vi "mupSetLocale.vi"(8 "error in (no error)":errorcluster, 10 "Use system decimal point (T)":bool=TRUE, 11 "hParser in":u64) -> (0 "error out":errorcluster, 3 "hParser out":u64)   [LabVIEW 2018, in "mupLib.lvlib"]
doc: "Set to true to use system's decimal point.\n\nIf the system's decimal point is a comma, the argument separator will be changed to a semi-colon.\n\nThe default decimal point is a period. The default argument separator is a comma."
uses:
  mupLib.lvlib
  libmuparser-lv.dll
panel:
  # "Set to true to use system's decimal point.\n\nIf the system's decimal point is a comma, the argument separator will be changed to a semi-colon.\n\nThe default decimal point is a period. The default argument separator is a comma."
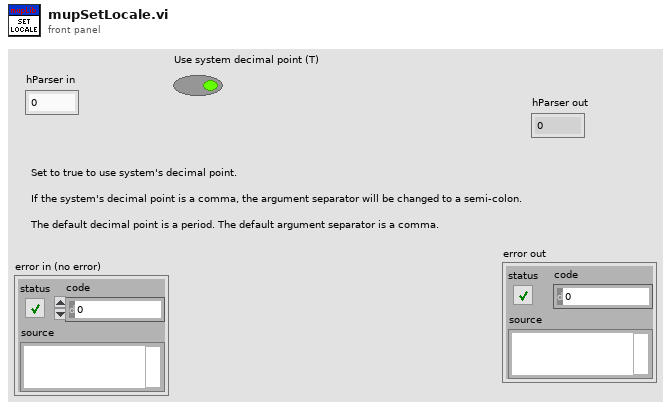
[diagram p1: front panel]
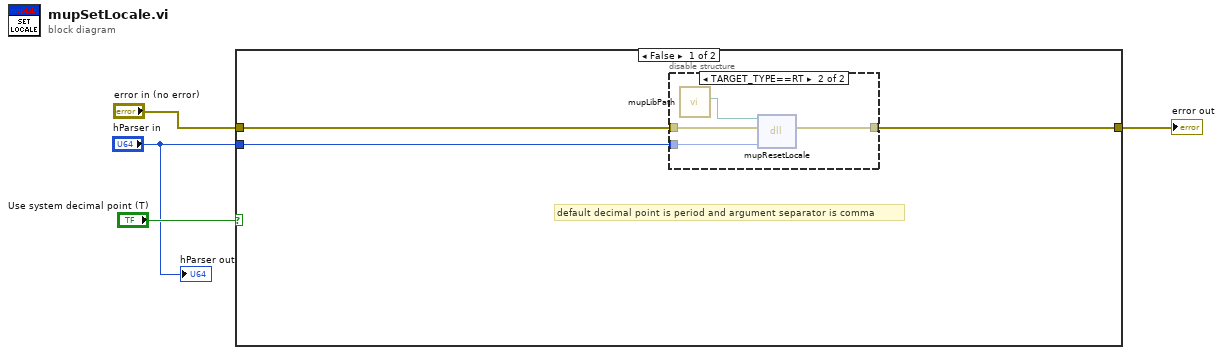
[diagram p0: block diagram]
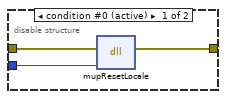
[diagram p2: hidden frame]
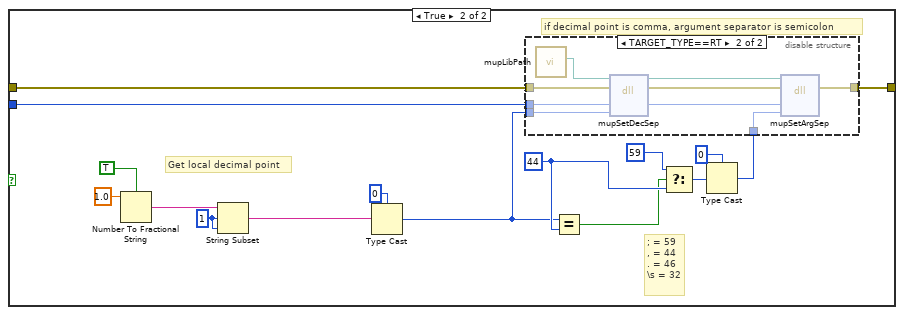
[diagram p3: hidden frame]
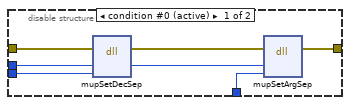
[diagram p4: hidden frame]
diagram:
  n1 = case shown="False" "Use system decimal point (T)" {
    tunnel: [w5 w30] -> w4
    tunnel: "error in (no error)" -> [w7 w21]
    tunnel: "hParser in" -> [w6 w22]
    frame False {
      # "default decimal point is period and argument separator is comma"
      n2 = disable-structure shown="TARGET_TYPE==RT" {
        disable-tunnel: w7 -> [w10 w14]
        disable-tunnel: w6 -> [w9 w13]
        disable-tunnel: [w8 w12] -> w5
        frame condition #0 (active) {
          n3 = dll-call lib="C:/Users/leonidas/Documents/GitHub/LV-muParser/mupLib/libmuparser-lv.dll" fn="mupResetLocale"(error in=w10, "hParser"=w9) -> (error out=w8:errorcluster)  [unwired: 4 in, 1 out]
        }
        frame condition #1 {
          n4 = call "mupLibPath.vi"() -> ("libmuparser path"=w11:path)  [unwired: 11 in]
          n5 = dll-call lib="C:/Users/leonidas/Documents/GitHub/LV-muParser/mupLib/libmuparser-lv.dll" fn="mupResetLocale"(path in=w11, error in=w14, "hParser"=w13) -> (error out=w12:errorcluster)  [unwired: 3 in, 1 out]
        }
      }
    }
    frame True {
      w16 = 1 ("offset (0)")
      w25 = u8 44 ("y")
      # "if decimal point is comma, argument separator is semicolon"
      # "Get local decimal point"
      # "; = 59\n, = 44\n. = 46\n\\s = 32"
      n6 = Number To Fractional String(use system decimal point (T)=TRUE, number=1.0) -> (F-format string=w17:string)  [unwired: 2 in]
      n7 = String Subset(string=w17, offset (0)=w16, length (rest)=w16) -> (substring=w15:string)
      n8 = Type Cast(type=u8 0, x=w15) -> (*(type *) &x=w23:u8)
      n9 = Equal?(x=w23, y=w25) -> (x = y?=w20:bool)
      n10 = Select(t=u8 59 ("y"), s=w20, f=w25) -> (s? t:f=w28:u8)
      n11 = Type Cast(type=u8 0, x=w28) -> (*(type *) &x=w27:u8)
      n12 = disable-structure shown="TARGET_TYPE==RT" {
        disable-tunnel: [w36 w45] -> w30
        disable-tunnel: w27 -> [w35 w44]
        disable-tunnel: w23 -> [w33 w42]
        disable-tunnel: w22 -> [w32 w41]
        disable-tunnel: w21 -> [w31 w40]
        frame condition #0 (active) {
          n13 = dll-call lib="C:/Users/leonidas/Documents/GitHub/LV-muParser/mupLib/libmuparser-lv.dll" fn="mupSetDecSep"(error in=w31, "hParser"=w32, "szChar"=w33) -> (error out=w37:errorcluster, "hParser"=w34:u64)  [unwired: 4 in, 1 out]
          n14 = dll-call lib="C:/Users/leonidas/Documents/GitHub/LV-muParser/mupLib/libmuparser-lv.dll" fn="mupSetArgSep"(error in=w37, "hParser"=w34, "szChar"=w35) -> (error out=w36:errorcluster)  [unwired: 5 in, 1 out]
        }
        frame condition #1 {
          n15 = call "mupLibPath.vi"() -> ("libmuparser path"=w39:path)  [unwired: 11 in]
          n16 = dll-call lib="C:/Users/leonidas/Documents/GitHub/LV-muParser/mupLib/libmuparser-lv.dll" fn="mupSetDecSep"(path in=w39, error in=w40, "hParser"=w41, "szChar"=w42) -> (path out=w38:path, error out=w46:errorcluster, "hParser"=w43:u64)  [unwired: 3 in]
          n17 = dll-call lib="C:/Users/leonidas/Documents/GitHub/LV-muParser/mupLib/libmuparser-lv.dll" fn="mupSetArgSep"(path in=w38, error in=w46, "hParser"=w43, "szChar"=w44) -> (error out=w45:errorcluster)  [unwired: 4 in, 1 out]
        }
      }
    }
  }
  "error out" <- w4
  "hParser out" <- "hParser in"
